vi "Route Error to Queue.vi"(8 "error in":errorcluster, 11 "Queue In":refnum<queue>) -> (0 "error out":errorcluster, 2 "Stop Loop?":bool, 3 "Queue Out":refnum<queue>)   [LabVIEW 2026]
doc: "Routes an error from a loop of Main.vi to the main message loop as an Error message, which that loop logs with Log Queued Error.vi. Wire it after a loop's case or event structure.\n\nerror in has no error (status FALSE, a warning included): Queue In is passed to Queue Out, error in is passed to error out unchanged and Stop Loop? is FALSE.\nerror in has error code 1, 1122 or 1556 (the queue refnum is invalid or was released): nothing is enqueued, Stop Loop? is TRUE and error out = error in.\nAny other error: Queue-Error.vi enqueues the error cluster as a variant (Message = Error, Data = the error cluster). If the enqueue succeeds, error out is clean and Stop Loop? is FALSE. If it fails, error out carries the enqueue error and Stop Loop? is TRUE.\n\nTerminals: Queue In and Queue Out - the internal message queue (element Messaging Cluster.ctl). error in and error out. Stop Loop? - TRUE when the calling loop should stop.\n\nDo NOT route the error of the main loop's own Error frame (an error from logging) back through this VI: every failed log would enqueue a new Error message and the loop would never end.\n\nGenerated by: Claude"
uses:
  Internal Message Library/Controls/Messaging Cluster.ctl
  Internal Message Library/Controls/Message.ctl
  Internal Message Library/Internal Messaging Library.lvlib
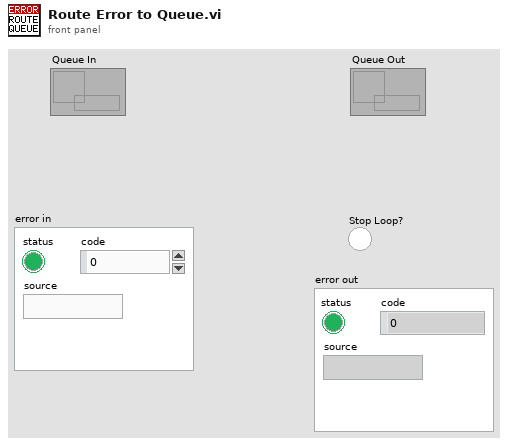
[diagram p1: front panel]
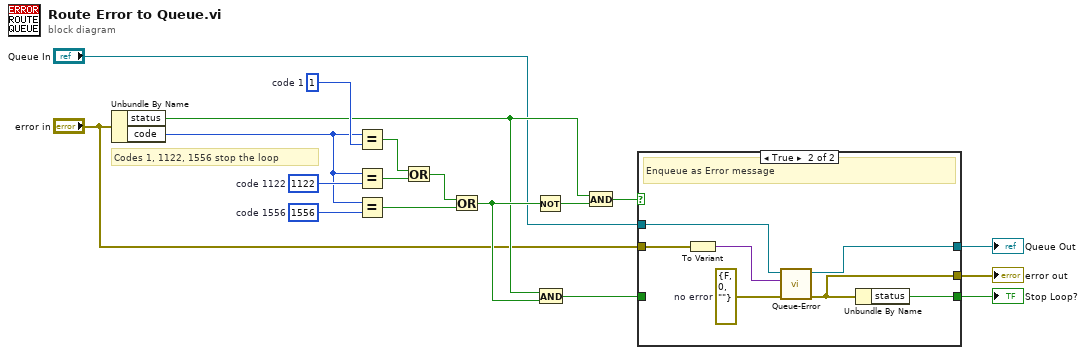
[diagram p0: block diagram]
diagram:
  w10 = 1556  # code 1556
  w9 = 1122  # code 1122
  w8 = 1  # code 1
  # "Codes 1, 1122, 1556 stop the loop"
  n1 = Unbundle By Name("error in") -> ("status"=w6:bool, "code"=w7:i32)
  n2 = Equal?(x=w7, y=w8) -> (x = y?=w11:bool)
  n3 = Equal?(x=w7, y=w9) -> (x = y?=w12:bool)
  n4 = Equal?(x=w7, y=w10) -> (x = y?=w13:bool)
  n5 = Or(x=w11, y=w12) -> (x .or. y?=w14:bool)
  n6 = Or(x=w14, y=w13) -> (x .or. y?=w15:bool)
  n7 = Not(x=w15) -> (.not. x?=w16:bool)
  n8 = And(x=w6, y=w15) -> (x .and. y?=w18:bool)
  n9 = And(x=w6, y=w16) -> (x .and. y?=w17:bool)
  n10 = case shown="True" w17 {
    tunnel: "Queue In" -> [w19 w22]
    tunnel: "error in" -> [w20 w23]
    tunnel: [w19 w26] -> w3
    tunnel: [w20 w27] -> w5
    tunnel: [w21 w28] -> w4
    tunnel: w18 -> [w21 _]
    frame False {
      # "Pass through"
    }
    frame True {
      w25 = errorcluster {"status"=FALSE, "code"=0, "source"=""}  # no error
      # "Enqueue as Error message"
      n11 = To Variant(anything=w23) -> (Variant=w24:variant)
      n12 = call "Queue-Error.vi"("error in"=w25, "Data"=w24, "Queue In"=w22) -> ("error out"=w27:errorcluster, "Queue Out"=w26:refnum<queue>)  [unwired: 7 in]
      n13 = Unbundle By Name(w27) -> ("status"=w28:bool)
    }
  }
  "Queue Out" <- w3
  "Stop Loop?" <- w4
  "error out" <- w5
